vi "create debug configuration.vi"() -> (0 "error out":errorcluster, 2 "mapping dvr":refnum<data-value>, 3 "engine dvr":refnum<data-value>)   [LabVIEW 2013, in "PL Framework Configuration Tool.lvlib" / "Engine Mappings.lvclass"]
uses:
  Engine Mappings.lvclass
  Engine Parent/Engine Parent Editor Node.lvclass
  <vilib>/NI/Module Execution Interface/Engine Configuration/engine configuration.lvclass
  <vilib>/NI/Configuration Framework/Node/NISE_CEF_Node.lvclass/NISE_CEF_Node.ctl
  <vilib>/NI/Configuration Framework/Node/ReadChildren.vi
  Engine Parent/write engine configuration.vi
  <vilib>/NI/Tag Bus/tag/tag descriptor.lvclass
  <vilib>/NI/Configuration Framework/Node/NISE_CEF_Node.lvclass
  <vilib>/NI/Tag Bus/tag/Data Type.ctl
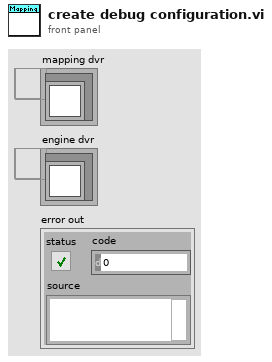
[diagram p1: front panel]
types:
  T1 = typedef "NISE_CEF_Node.lvclass/NodeRef.ctl" = refnum<data-value>
  T2 = typedef "tag bus.lvlib/tag descriptor.lvclass/Data Type.ctl" = enum16{"Double", "Single", "I64", "I32", "I16", "I8", "U64", "U32", "U16", "U8", "Boolean", "String", "Array of Double", "Array of Single", "Array of I64", "Array of I32", "Array of I16", "Array of I8", "Array of U64", "Array of U32", "Array of U16", "Array of U8", "Array of Boolean", "Array of String"}
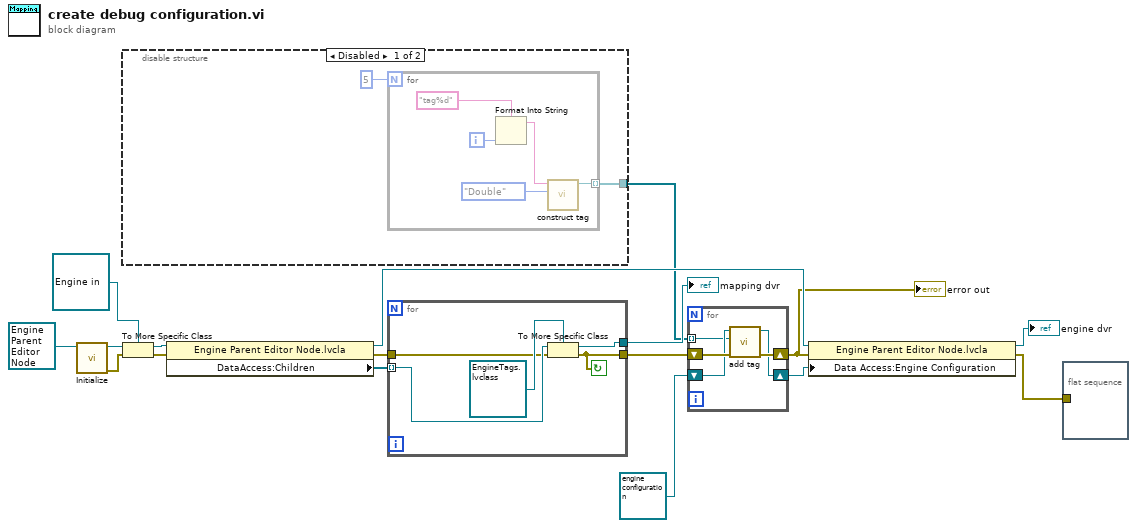
[diagram p0: block diagram]
diagram:
  n1 = call-dynamic "Initialize.vi"("Engine in"=refnum<class "Engine Parent Editor Node.lvclass"> refnum) -> ("error out"=w16:errorcluster, "data value reference"=w13:T1)  [unwired: 8 in, 1 out]
  n2 = disable-structure shown="Disabled" {
    disable-tunnel: [w18 _] -> w6
    frame Disabled {
      n3 = for {
        N: 5 -> [_]
        tunnel: [w20] -> w18 mode=indexing
        i -> [w24]
        n4 = Format Into String(format string="tag%d", w24) -> (resulting string=w22:string)  [unwired: 2 in, 1 out]
        n5 = call <vilib>:"construct tag.vi"("data type"=Data_Type."Double", "name"=w22) -> ("system tag out"=w20:refnum<class "tag descriptor.lvclass">)  [unwired: 8 in, 1 out]
      }
    }
    frame Enabled {
    }
  }
  n6 = To More Specific Class(target class=refnum<data-value> refnum ("data value reference"), reference=w13, error in=w16) -> (specific class reference=w12:refnum<data-value>, error out=w15:errorcluster)
  n7 = property class="Engine Parent Editor Node.lvcla"(reference=w12, error in=w15) -> (reference out=w8:refnum<data-value>, error out=w5:errorcluster, "DataAccess:Children"=w9:T1[])
  n8 = for {
    tunnel: [w26] -> w17
    tunnel: [w28] -> w14
    tunnel: w9 -> [w27] mode=indexing
    tunnel: w5 -> [w25]
    stop <- w26 continue-if-true
    n9 = To More Specific Class(target class=refnum<data-value> refnum ("data value reference"), reference=w27, error in=w25) -> (specific class reference=w28:refnum<data-value>, error out=w26:errorcluster)
  }
  "mapping dvr" <- w14
  n10 = for {
    shift-right: [w32] -> w3
    shift-left: refnum<class "engine configuration.lvclass"> refnum ("engine configuration.lvclass") -> [w31]
    shift-right: [w34] -> w2
    shift-left: w17 -> [w33]
    tunnel: w6 -> [w30] mode=indexing
    n11 = call <vilib>:"add tag.vi"("error in"=w33, "tag descriptor"=w30, "engine configuration in"=w31) -> ("error out"=w34:errorcluster, "engine configuration out"=w32:refnum<class "engine configuration.lvclass">)  [unwired: 7 in]
  }
  "error out" <- w2
  n12 = property class="Engine Parent Editor Node.lvcla"(reference=w8, error in=w2, "Data Access:Engine Configuration"=w3) -> (reference out=→"engine dvr":refnum<data-value>, error out=w1:errorcluster)
  n13 = flat-sequence {
    tunnel: w1 -> [_]
    frame #0 {
    }
  }
